vi "Query_MP.vi"(5 "buffered":bool=TRUE, 6 "commandTimeout":i32=-1, 7 "CommandType":i32(ring)=-1 items=["Text"=1, "StoredProcedure"=4, "TableDirect"=512], 8 "error in (no error)":errorcluster, 9 "DynamicParameters":refnum<class "DynamicParameters.lvclass">[](array[class]), 10 "sql":string, 11 "ADOMapper in":refnum<class "ADOMapper.lvclass">) -> (0 "error out":errorcluster, 2 "Query Result out":refnum<class "Query Result.lvclass">, 3 "ADOMapper out":refnum<class "ADOMapper.lvclass">)   [LabVIEW 2026, in "ORM_ADONetCore.lvlib" / "ADOMapper.lvclass"]
uses:
  ADOMapper.lvclass
  <vilib>/Viviota/shared/ORM.lvlibp/Query Result/Query Result.lvclass
  <vilib>/Viviota/shared/ORM.lvlibp/DynamicParameters/DynamicParameters.lvclass
  <vilib>/Viviota/shared/ORM_DBC_dotNetCore.lvlibp/ORM_DBC_dotNetCore.lvclass
  ADOResult/ADOResult.lvclass
  <vilib>/Viviota/shared/ORM.lvlibp/SqlMapper/Read DbConnection.vi
  <vilib>/Viviota/shared/ORM_DBC_dotNetCore.lvlibp/Read transaction.vi
  C:/Program Files/dotnet/shared/Microsoft.NETCore.App/8.0.28/System.Data.Common.dll
  Program Files/dotnet/shared/Microsoft.NETCore.App/8.0.28/System.Data.Common.dll
  <vilib>/Viviota/shared/ORM.lvlibp/DbConnection/DbConnection.lvclass
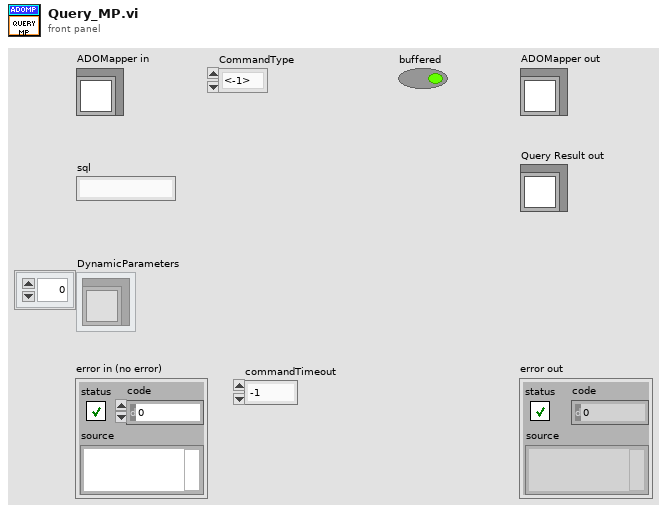
[diagram p1: front panel]
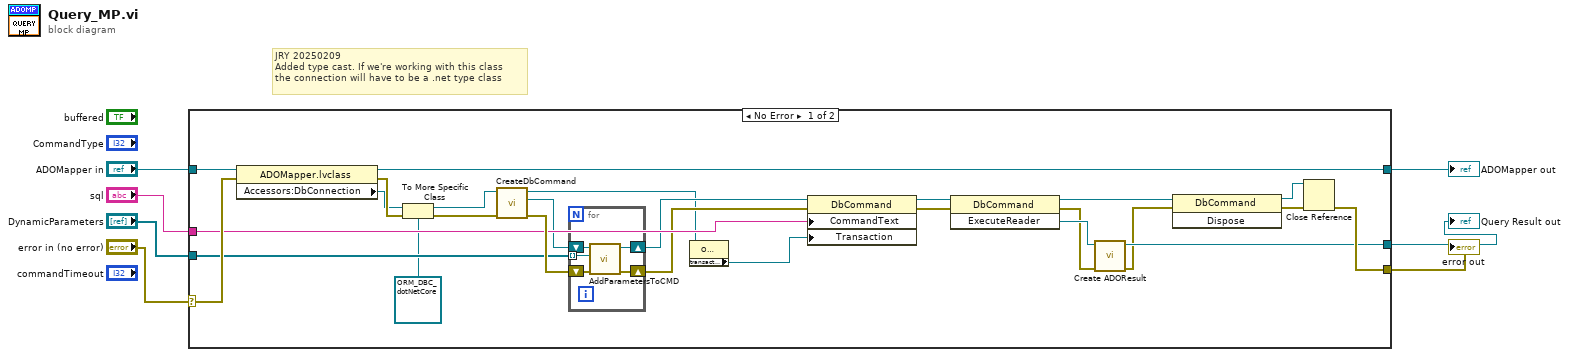
[diagram p0: block diagram]
diagram:
  # "JRY 20250209\nAdded type cast. If we're working with this class\nthe connection will have to be a .net type class"
  n1 = case shown="No Error" "error in (no error)" {
    selector: "error in (no error)" -> [w31 w40]
    tunnel: "ADOMapper in" -> [w33 w39]
    tunnel: [w32 w39] -> w6
    tunnel: "sql" -> [w28 _]
    tunnel: [w22 w40] -> w1
    tunnel: "DynamicParameters" -> [w19 _]
    tunnel: [w17 _] -> w5
    frame No Error {
      n2 = property class="ADOMapper.lvclass"(reference=w33, error in=w31) -> (reference out=w32:refnum<class "ADOMapper.lvclass">, error out=w30:errorcluster, "Accessors:DbConnection"=w10:refnum<class "DbConnection.lvclass">)
      n3 = To More Specific Class(target class=refnum<class "ORM_DBC_dotNetCore.lvclass"> refnum ("ORM_DBC_dotNetCore.lvlibp:ORM_DBC_dotNetCore.lvclass"), reference=w10, error in=w30) -> (specific class reference=w9:refnum<class "ORM_DBC_dotNetCore.lvclass">, error out=w11:errorcluster)
      n4 = call <vilib>:"CreateDbCommand.vi"("error in (no error)"=w11, "DbConnection in"=w9) -> ("error out"=w29:errorcluster, "Command"=w20:refnum<k39>, "DbConnection out"=w13:refnum<class "ORM_DBC_dotNetCore.lvclass">)  [unwired: 7 in]
      n5 = for {
        tunnel: w19 -> [w35] mode=indexing
        shift-right: [w37] -> w26
        shift-left: w29 -> [w38]
        shift-right: [w34] -> w18
        shift-left: w20 -> [w36]
        n6 = call "AddParametersToCMD.vi"("error in (no error)"=w38, "DynamicParameters in"=w35, "CreateCommand"=w36) -> ("error out"=w37:errorcluster, "Command Out"=w34:refnum<k39>)  [unwired: 7 in]
      }
      n7 = property class="ORM_DBC_dotNetCore.lvclass"(reference=w13) -> ("transaction"=w12:refnum<k39>)  [unwired: 1 in, 2 out]
      n8 = property class="DbCommand"(reference=w18, error in=w26, "CommandText"=w28, "Transaction"=w12) -> (reference out=w27:refnum<k39>, error out=w25:errorcluster)
      n9 = invoke class="DbCommand" method="ExecuteReader"(reference=w27, error in=w25) -> (reference out=w24:refnum<k39>, error out=w15:errorcluster, "ExecuteReader"=w16:refnum<k39>)  [unwired: 1 in]
      n10 = call "Create ADOResult.vi"("error in (no error)"=w15, "Reader"=w16) -> ("error out"=w14:errorcluster, "ADOResult out"=w17:refnum<class "ADOResult.lvclass">)  [unwired: 8 in]
      n11 = invoke class="DbCommand" method="Dispose"(reference=w24, error in=w14) -> (reference out=w21:refnum<k39>, error out=w23:errorcluster)  [unwired: 1 in, 1 out]
      n12 = Close Reference(reference=w21, error in (no error)=w23) -> (error out=w22:errorcluster)
    }
    frame Error {
    }
  }
  "error out" <- w1
  "ADOMapper out" <- w6
  "Query Result out" <- w5
